vi "GOOPUtil_IsValidReference.vi"(0 "LabVIEW Object":refnum<class>, 5 "error in (no error)":errorcluster) -> (14 "Not a refnum?":bool, 15 "Class Name":string, 19 "error out":errorcluster)   [LabVIEW 2020, in "GOOPUtility.lvlib"]
doc: "Checks if a reference contains a valid GOOP reference.\n\nThis is a collection of generic GOOP utility VIs. Please notice that it is important that the frontpanel of the Create, Destroy and GetObjectStatus is not removed when building an application."
uses:
  GOOPUtility.lvlib
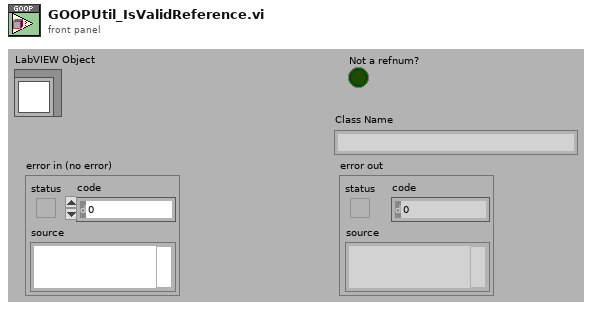
[diagram p1: front panel]
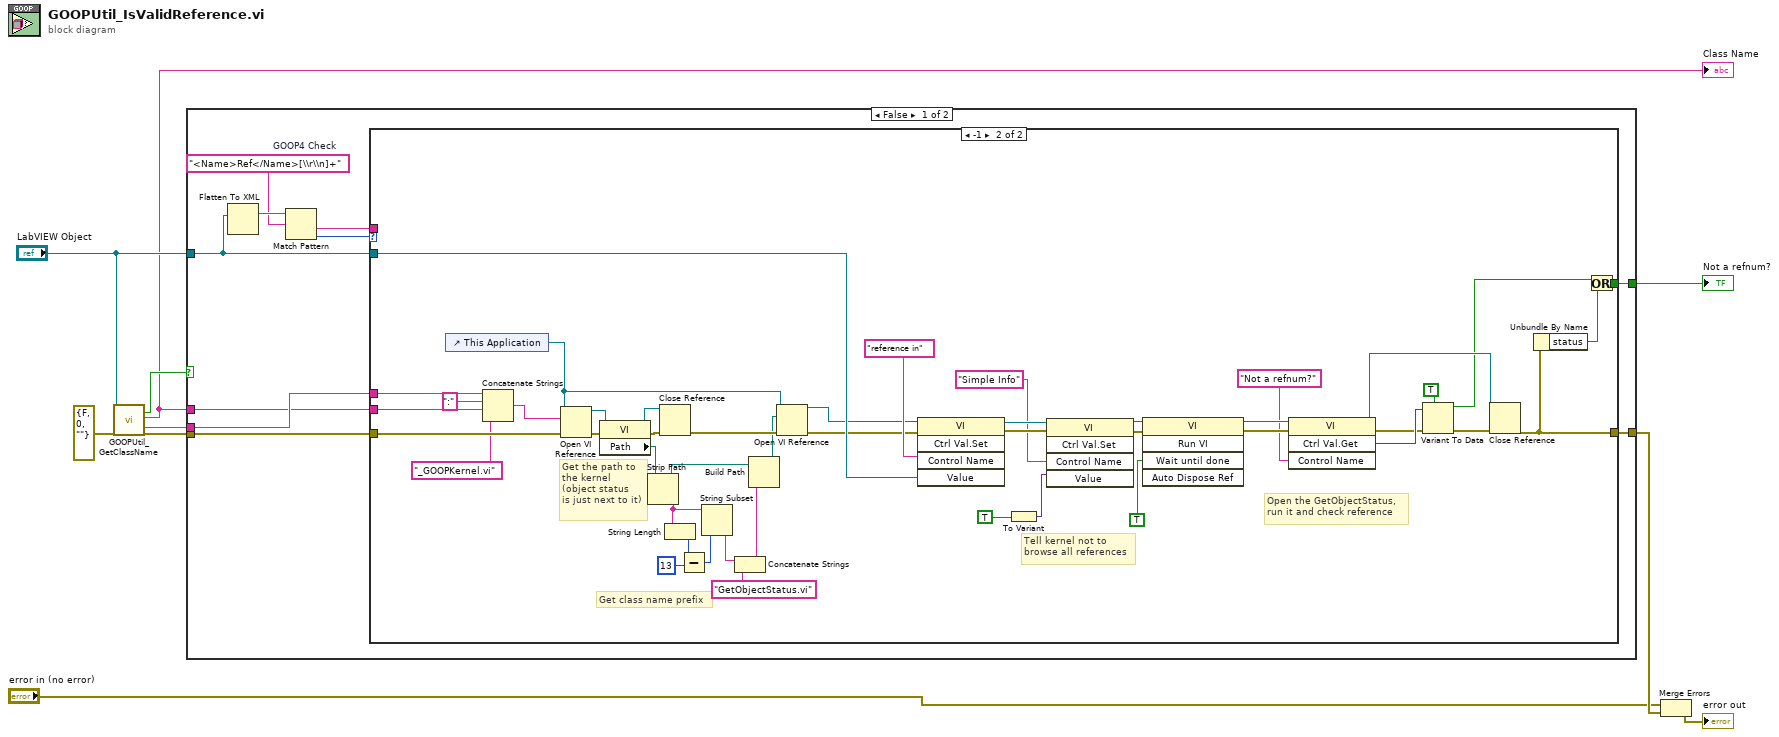
[diagram p0: block diagram]
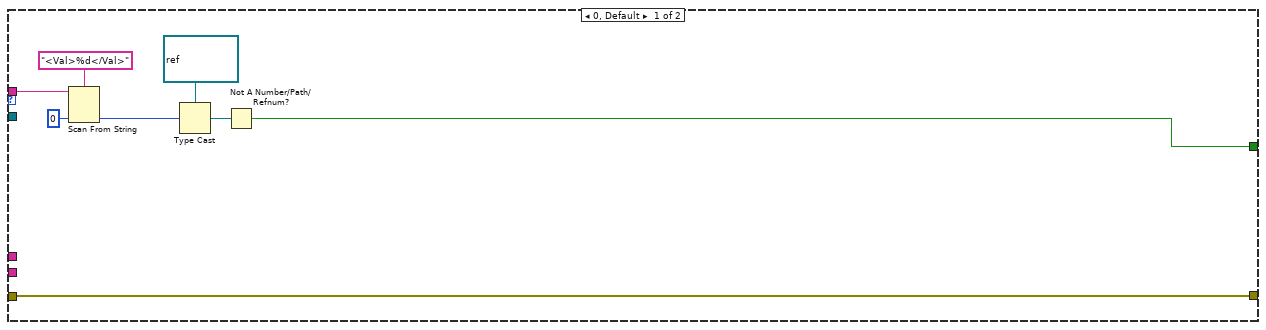
[diagram p2: hidden frame]
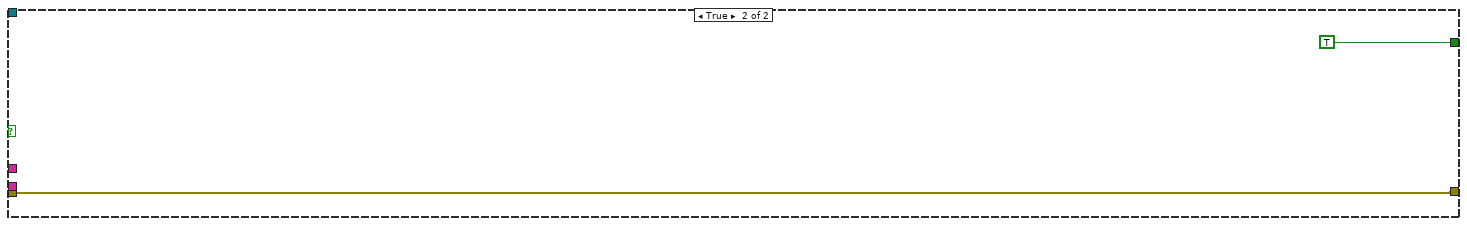
[diagram p3: hidden frame]
diagram:
  n1 = call "GOOPUtil_GetClassName.vi"("LabVIEW Object"="LabVIEW Object", "error in (no error)"=errorcluster {"status"=FALSE, "code"=0, "source"=""}) -> ("IsEmptyObject?"=w9:bool, "Class Name"=w1:string, "Full Class Name"=w2:string, "error out"=w8:errorcluster)  [unwired: 13 in, 1 out]
  "Class Name" <- w1
  n2 = case shown="False" w9 {
    tunnel: "LabVIEW Object" -> [w15 _]
    tunnel: w8 -> [w18 w75]
    tunnel: [w20 TRUE] -> w6
    tunnel: [w19 w75] -> w4
    tunnel: w2 -> [w17 _]
    tunnel: w1 -> [w16 _]
    frame False {
      w13 = "<Name>Ref</Name>[\\r\\n]+"  # GOOP4 Check
      n3 = Flatten To XML(6:w15) -> (2:w14:string)
      n4 = Match Pattern(string=w14, regular expression=w13) -> (after substring=w11:string, offset past match=w12:i32)  [unwired: 1 in, 2 out]
      n5 = case shown="-1" w12 {
        tunnel: [w22 w52] -> w20
        tunnel: [w21 w39] -> w19
        tunnel: w18 -> [w21 w38]
        tunnel: w17 -> [_ w37]
        tunnel: w16 -> [_ w35]
        tunnel: w15 -> [_ w31]
        tunnel: w11 -> [w28 _]
        frame 0, Default {
          n6 = Scan From String(format string="<Val>%d</Val>", input string=w28, default 1=u32 0 ("default value 1")) -> (output 1=w26:u32)  [unwired: 2 in, 3 out]
          n7 = Type Cast(type=refnum<data-value> refnum ("data value reference"), x=w26) -> (*(type *) &x=w23:refnum<data-value>)
          n8 = Not A Number/Path/Refnum?(number/path/refnum=w23) -> (NaN/Path/Refnum?=w22:bool)
        }
        frame -1 {
          # "Tell kernel not to\nbrowse all references"
          # "Open the GetObjectStatus,\nrun it and check reference"
          # "Get the path to\nthe kernel\n(object status\nis just next to it)"
          # "Get class name prefix"
          n9 = control-ref of="This Application"() -> (w33:refnum<vi>)
          n10 = Concatenate Strings(w37, ":" ("string"), w35, "_GOOPKernel.vi") -> (w32:string)
          n11 = Open VI Reference(application reference (local)=w33, vi path=w32, error in (no error)=w38) -> (vi reference=w73:refnum<vi>, error out=w74:errorcluster)  [unwired: 3 in]
          n12 = property class="VI"(reference=w73, error in=w74) -> (reference out=w71:refnum<vi>, error out=w72:errorcluster, "Path"=w69:path)
          n13 = Strip Path(path=w69) -> (stripped path=w59:path, name=w65:string)
          n14 = Close Reference(reference=w71, error in (no error)=w72) -> (error out=w70:errorcluster)
          n15 = String Length(string=w65) -> (length=w68:i32)
          n16 = Subtract(x=w68, y=13) -> (x-y=w66:i32)
          n17 = String Subset(string=w65, length (rest)=w66) -> (substring=w60:string)  [unwired: 1 in]
          n18 = Concatenate Strings(w60, "GetObjectStatus.vi") -> (w63:string)
          n19 = Build Path(base path=w59, name or relative path=w63) -> (appended path=w62:path)
          n20 = Open VI Reference(application reference (local)=w33, vi path=w62, error in (no error)=w70) -> (vi reference=w29:refnum<vi>, error out=w30:errorcluster)  [unwired: 3 in]
          n21 = invoke class="VI" method="Ctrl Val.Set"(reference=w29, error in=w30, "Control Name"="reference in", "Value"=w31) -> (reference out=w50:refnum<vi>, error out=w51:errorcluster)  [unwired: 1 in, 3 out]
          n22 = To Variant(anything=TRUE ("Wait Until Done")) -> (Variant=w40:variant)
          n23 = invoke class="VI" method="Ctrl Val.Set"(reference=w50, error in=w51, "Control Name"="Simple Info", "Value"=w40) -> (reference out=w48:refnum<vi>, error out=w49:errorcluster)  [unwired: 1 in, 3 out]
          n24 = invoke class="VI" method="Run VI"(reference=w48, error in=w49, "Wait until done"=TRUE ("Wait Until Done")) -> (reference out=w56:refnum<vi>, error out=w57:errorcluster)  [unwired: 2 in, 3 out]
          n25 = invoke class="VI" method="Ctrl Val.Get"(reference=w56, error in=w57, "Control Name"="Not a refnum?") -> (reference out=w54:refnum<vi>, error out=w45:errorcluster, "Get Control Value Variant"=w46:variant)  [unwired: 1 in, 1 out]
          n26 = Variant To Data(error in=w45, type=TRUE, Variant=w46) -> (data=w42:bool, error out=w44:errorcluster)
          n27 = Close Reference(reference=w54, error in (no error)=w44) -> (error out=w39:errorcluster)
          n28 = Unbundle By Name(w39) -> ("status"=w53:bool)
          n29 = Or(x=w42, y=w53) -> (x .or. y?=w52:bool)
        }
      }
    }
    frame True {
    }
  }
  "Not a refnum?" <- w6
  n30 = Merge Errors("error in (no error)", w4) -> (→"error out":errorcluster)
